vi "ReadAOs.vi"(8 "error in (no error)":errorcluster, 10 "Analog Output":T2, 11 "VISA resource name":refnum<visa-resource-name>) -> (0 "error out":errorcluster, 2 "AnOutValues":T1, 3 "VISA resource name out":refnum<visa-resource-name>)   [LabVIEW 2020, in "HandsOnPi2040.lvlib"]
uses:
  HandsOnPi2040.lvlib
  cti-drivers-lv-visa-main/CTI-Visa/CTI-Visa.lvlib
  PWMSettings.ctl
  AOs.ctl
panel:
  # "Output"
  # "Input"
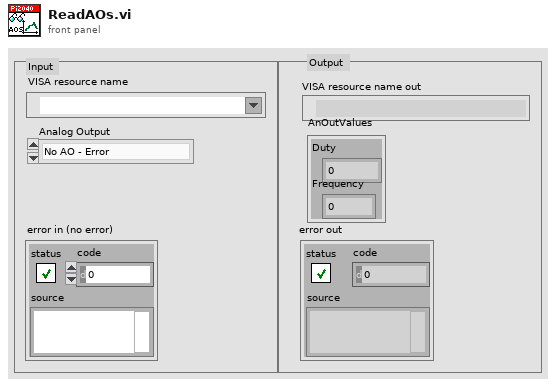
[diagram p1: front panel]
types:
  T1 = typedef "HandsOnPi2040.lvlib/PWMSettings.ctl" = cluster{"Duty":sgl, "Frequency":sgl}
  T2 = typedef "HandsOnPi2040.lvlib/AOs.ctl" = enum16{"No AO - Error", "AO1 (GPIO28)"}
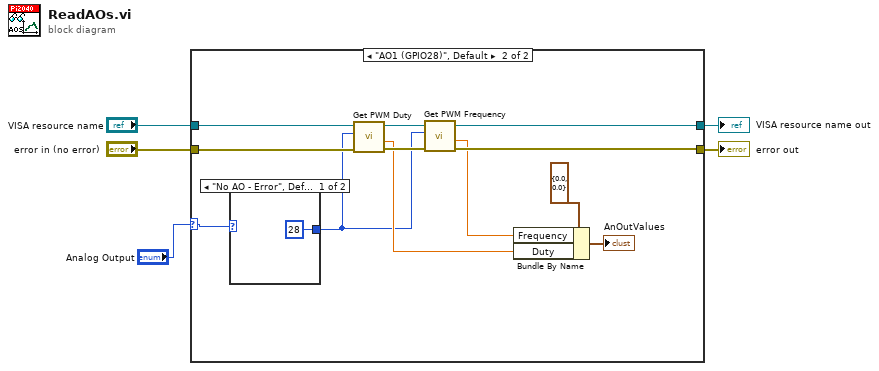
[diagram p0: block diagram]
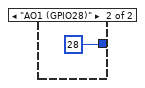
[diagram p3: hidden frame]
diagram:
  n1 = case shown="\"AO1 (GPIO28)\", Default" "Analog Output" {
    selector: "Analog Output" -> [_ w9]
    tunnel: "VISA resource name" -> [w6 w19]
    tunnel: "error in (no error)" -> [w7 w18]
    tunnel: [w6 w12] -> w5
    tunnel: [w7 w13] -> w4
    frame "No AO - Error" {
    }
    frame "AO1 (GPIO28)", Default {
      n2 = case shown="\"No AO - Error\", Default" w9 {
        tunnel: [28 ("Channel") 28 ("Channel")] -> w8
        frame "No AO - Error", Default {
        }
        frame "AO1 (GPIO28)" {
        }
      }
      n3 = call "Get PWM Duty.vi"("error in (no error)"=w18, "Channel"=w8, "VISA resource name in"=w19) -> ("error out"=w14:errorcluster, "Duty % (0-1)"=w10:sgl, "VISA resource name"=w15:refnum<visa-resource-name>)  [unwired: 6 in]
      n4 = call "Get PWM Frequency.vi"("error in (no error)"=w14, "Channel"=w8, "VISA resource name in"=w15) -> ("error out"=w13:errorcluster, "Freq Hz"=w11:sgl, "VISA resource name"=w12:refnum<visa-resource-name>)  [unwired: 6 in]
      n5 = Bundle By Name(cluster=T1 {"Duty"=0.0, "Frequency"=0.0} ("AnOutValues"), "Frequency"=w11, "Duty"=w10) -> (→"AnOutValues":T1)
    }
  }
  "VISA resource name out" <- w5
  "error out" <- w4
